vi "[ex ce] Handling Custom Data Types.vi"() -> ()   [LabVIEW 2021]
doc: "<B>Variable Manager example</B>\n\nThe VI demonstrates how to use user-defined data types with Variable Manager.\n\nThe VI generates a LabVIEW Waveform and saves it in a VarMan variable. The variable has a history attached, which saves every value written to the variable.\n\nThe example VI reads the variable to indicate current Waveform generated. Furthermore, it reads the variable history to indicate Waveforms generated recently.\n\n::: CalcExpress Toolkit :::\nCopyright (c) 2000-2026 Konstantin Shifershteyn. All rights reserved."
uses:
  <vilib>/measure/NI_MAPro.lvlib
panel:
  out "writerID":u32
  in  "tone phases":dbl[](array[numeric])=[137.63, 330.58, 66.37, 301.58] format="%.2p"
  in  "tone amplitudes":dbl[](array[numeric])=[2.0, 1.0, 1.0, 1.0] format="%.2p"
  in  "tone frequencies":dbl[](array[numeric])=[4.0, 2.0, 10.0, 8.0] format="%.2p"
  out "Timestamp":dbl format="%<%H:%M:%S%3u\n%x>T"
  in  "Hist Idx":i32(slide) caption="Historic point index" scale=0.0..99.0
  in  "Read History":bool
  out "Historic Graph":waveform(dbl)(graph)
  in  "stop":bool
  out "Waveform Graph":waveform(dbl)(graph)
  # "Review description for this VI and its Block Diagram for details"
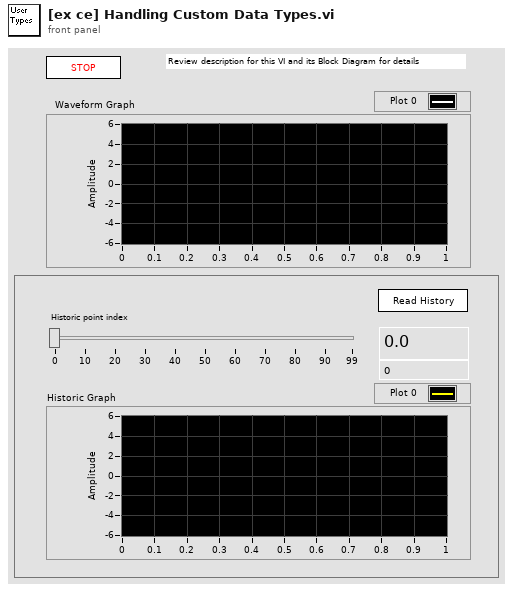
[diagram p1: front panel]
types:
  T1 = enum32{"nop", "create", "destroy", "reset", "get info", "config", "create_wrid"}
  T2 = typedef "VarMan Variable Context Handle.ctl" = i32
  T3 = enum8{"Enabled", "Disabled", "Disabled and Grayed Out"}
  T4 = typedef "VarMan Variable Data Statistics.ctl" = cluster{"writer ID":u32, "write MS":u32, "write TS":dbl, "write Cnt":u32}
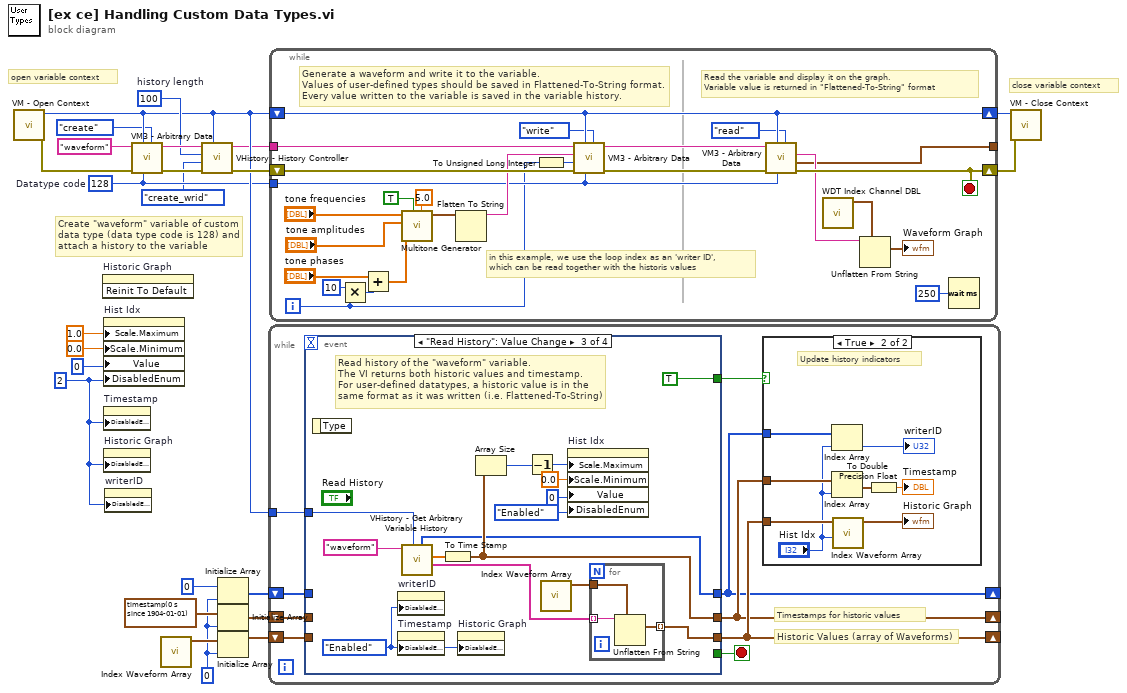
[diagram p0: block diagram]
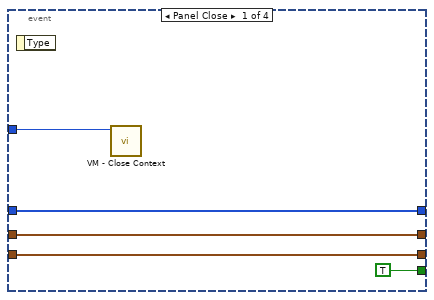
[diagram p3: hidden frame]
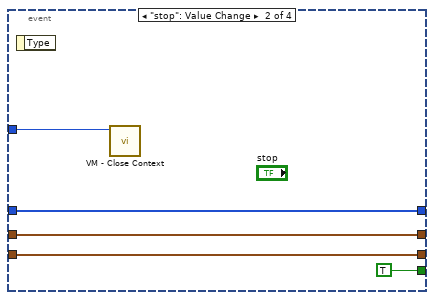
[diagram p4: hidden frame]
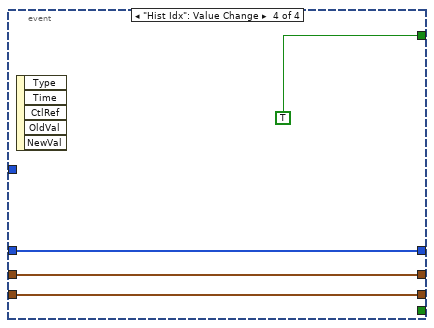
[diagram p5: hidden frame]
diagram:
  w4 = 0
  w19 = 100  # history length
  w1 = u8 2 ("Disabled")
  w14 = u32 128  # Datatype code
  # "close variable context"
  # "open variable context"
  # "Create \"waveform\" variable of custom\ndata type (data type code is 128) and\nattach a history to the variable"
  n1 = call "VM - Open Context.vi"() -> ("error out"=w23:errorcluster, "VC Handle out"=w16:T2)  [unwired: 9 in, 1 out]
  n2 = invoke on="Historic Graph" class="WFGraph (strict)" method="Reinit To Default"() -> ()  [unwired: 3 in, 3 out]
  n3 = property on="Hist Idx" class="Slide (strict)"("Scale.Maximum"=1.0 ("Scale.Range:Maximum"), "Scale.Minimum"=0.0 ("Scale.Range:Minimum"), "Value"=0 ("Slide"), "DisabledEnum"=w1) -> ()  [unwired: 2 in, 2 out]
  n4 = property on="Timestamp" class="DigNum (strict)"("DisabledEnum"=w1) -> ()  [unwired: 2 in, 2 out]
  n5 = property on="Historic Graph" class="WFGraph (strict)"("DisabledEnum"=w1) -> ()  [unwired: 2 in, 2 out]
  n6 = property on="writerID" class="DigNum (strict)"("DisabledEnum"=w1) -> ()  [unwired: 2 in, 2 out]
  n7 = call "VM3 - Arbitrary Data.vi"("cmd (read)"=enum16{"create", "destroy", "write", "read"}."create", "var type in"=w14, "VC Handle"=w16, "error in"=w23, "name_spec"="waveform" ("name")) -> ("error out"=w24:errorcluster, "dup name_spec"=w21:string)  [unwired: 2 in, 3 out]
  n8 = call-poly <vilib>:"Index Waveform Array.vi"() -> ("waveform"=w7:waveform(dbl))  [unwired: 10 in, 1 out]
  n9 = call "VHistory - History Controller.vi"("VC Handle"=w16, "error in"=w24, "cmd (nop:default)"=T1."create_wrid", "history length"=w19, "name_spec"=w21) -> ("error out"=w20:errorcluster, "dup name_spec"=w15:string)  [unwired: 3 in, 2 out]
  n10 = Initialize Array(u32 0, w4) -> (w3:u32[])
  n11 = Initialize Array(timestamp(0 s since 1904-01-01), w4) -> (w12:timestamp[])
  n12 = Initialize Array(w7, w4) -> (w13:waveform(dbl)[])
  n13 = while {
    tunnel: w16 -> [w33]
    shift-right: [w28] -> _
    shift-left: w13 -> [w32]
    shift-right: [w27] -> _
    shift-left: w12 -> [w31]
    shift-right: [w25] -> _
    shift-left: w3 -> [w26]
    stop <- w30 stop-if-true
    # "Timestamps for historic values"
    # "Historic Values (array of Waveforms)"
    n14 = event shown="[2] \"Read History\": Value Change" {
      selector: _ -> [_ _ _ _]
      dyn-events: _ -> [_ _ _ _]
      timeout: _ -> [_ _ _ _]
      tunnel: w33 -> [w44 w49 w66 _]
      tunnel: [w45 w50 w64 w73] -> w28
      tunnel: [w46 w51 w56 w72] -> w27
      tunnel: w32 -> [w45 w50 _ w73]
      tunnel: w31 -> [w46 w51 _ w72]
      tunnel: [TRUE TRUE _ _] -> w30
      tunnel: [_ _ TRUE TRUE] -> w29
      tunnel: [w42 w47 w53 w70] -> w25
      tunnel: w26 -> [w42 w47 _ w70]
      event Panel Close {
        n15 = event-data() -> ()  [unwired: 1 in, 1 out]
        n16 = call "VM - Close Context.vi"("VC Handle"=w44) -> ()  [unwired: 9 in, 2 out]
      }
      event "stop": Value Change {
        n17 = event-data() -> ()  [unwired: 1 in, 1 out]
        n18 = call "VM - Close Context.vi"("VC Handle"=w49) -> ()  [unwired: 9 in, 2 out]
      }
      event "Read History": Value Change {
        w52 = T3."Enabled" ("Disabled")
        # "Read history of the \"waveform\" variable.\nThe VI returns both historic values and timestamp.\nFor user-defined datatypes, a historic value is in the\nsame format as it was written (i.e. Flattened-To-String)"
        n19 = event-data() -> ()  [unwired: 1 in, 1 out]
        n20 = property on="writerID" class="DigNum (strict)"("DisabledEnum"=w52) -> ()  [unwired: 2 in, 2 out]
        n21 = property on="Timestamp" class="DigNum (strict)"("DisabledEnum"=w52) -> ()  [unwired: 2 in, 2 out]
        n22 = call "VHistory - Get Arbitrary Variable History.vi"("VC Handle"=w66, "name_spec"="waveform" ("name")) -> ("history"=w65:string[], "time stamps"=w63:dbl[], "writer IDs"=w53:u32[])  [unwired: 5 in, 2 out]
        n23 = To Time Stamp(1:w63) -> (0:w56:timestamp[])
        n24 = property on="Historic Graph" class="WFGraph (strict)"("DisabledEnum"=w52) -> ()  [unwired: 2 in, 2 out]
        n25 = Array Size(array=w56) -> (size(s)=w62:i32)
        n26 = Decrement(x=w62) -> (x-1=w58:i32)
        n27 = call-poly <vilib>:"Index Waveform Array.vi"() -> ("waveform"=w54:waveform(dbl))  [unwired: 10 in, 1 out]
        n28 = property on="Hist Idx" class="Slide (strict)"("Scale.Maximum"=w58, "Scale.Minimum"=0.0 ("Scale.Range:Minimum"), "Value"=0 ("Slide"), "DisabledEnum"=T3."Enabled" ("Disabled")) -> ()  [unwired: 2 in, 2 out]
        n29 = for {
          tunnel: w65 -> [w69] mode=indexing
          tunnel: w54 -> [w68]
          tunnel: [w67] -> w64 mode=indexing
          n30 = Unflatten From String(type=w68, binary string=w69) -> (value=w67:waveform(dbl))  [unwired: 3 in, 2 out]
        }
      }
      event "Hist Idx": Value Change {
        n31 = event-data() -> ()  [unwired: 1 in, 5 out]
      }
    }
    n32 = case shown="True" w29 {
      tunnel: w28 -> [_ w38]
      tunnel: w27 -> [_ w41]
      tunnel: w25 -> [_ w35]
      frame False {
      }
      frame True {
        # "Update history indicators"
        n33 = Index Array(array=w35, index="Hist Idx") -> (element=→"writerID":u32)
        n34 = Index Array(array=w41, index="Hist Idx") -> (element=w40:timestamp)
        n35 = call-poly <vilib>:"Index Waveform Array.vi"("index"="Hist Idx", "waveform array"=w38) -> ("waveform"=→"Historic Graph":waveform(dbl))  [unwired: 8 in, 1 out]
        n36 = To Double Precision Float(number=w40) -> (double precision float=→"Timestamp":dbl)
      }
    }
  }
  n37 = while {
    tunnel: w15 -> [w98]
    tunnel: w14 -> [w82]
    shift-right: [w85] -> w17
    shift-left: w20 -> [w97]
    shift-right: [w84] -> w18
    shift-left: w16 -> [w84]
    tunnel: [w76] -> _
    i -> [w75]
    stop <- w85 stop-if-true
    # "in this example, we use the loop index as an 'writer ID',\nwhich can be read together with the historis values"
    # "Read the variable and display it on the graph.\nVariable value is returned in \"Flattened-To-String\" format"
    # "Generate a waveform and write it to the variable.\nValues of user-defined types should be saved in Flattened-To-String format.\nEvery value written to the variable is saved in the variable history."
    n38 = Multiply(x=10, y=w75) -> (x*y=w89:i32)
    n39 = Add(x="tone phases", y=w89) -> (x+y=w91:dbl[])
    n40 = call <vilib>:"Multitone Generator.vi"("amplitude"=5.0, "reset signal"=TRUE, "tone phases"=w91, "tone amplitudes"="tone amplitudes", "tone frequencies"="tone frequencies") -> ("signal out"=w87:waveform(dbl))  [unwired: 3 in, 3 out]
    n41 = Flatten To String(anything=w87) -> (data string=w96:string)  [unwired: 3 in, 2 out]
    n42 = To Unsigned Long Integer(number=w75) -> (unsigned 32bit integer=w74:u32)
    n43 = call "VM3 - Arbitrary Data.vi"("cmd (read)"=enum16{"create", "destroy", "write", "read"}."write", "var type in"=w82, "VC Handle"=w84, "error in"=w97, "writer ID"=w74, "flattened value in"=w96, "name_spec"=w98) -> ("error out"=w86:errorcluster, "dup name_spec"=w83:string)  [unwired: 3 out]
    n44 = call "VM3 - Arbitrary Data.vi"("cmd (read)"=enum16{"create", "destroy", "write", "read"}."read", "var type in"=w82, "VC Handle"=w84, "error in"=w86, "name_spec"=w83) -> ("error out"=w85:errorcluster, "stats"=w76:T4, "flattened value out"=w81:string)  [unwired: 2 in, 2 out]
    n45 = call <vilib>:"WDT Index Channel DBL.vi"() -> ("waveform"=w80:waveform(dbl))  [unwired: 10 in, 1 out]
    n46 = Unflatten From String(type=w80, binary string=w81) -> (value=→"Waveform Graph":waveform(dbl))  [unwired: 3 in, 2 out]
    n47 = Wait (ms)(milliseconds to wait=u32 250) -> ()  [unwired: 1 out]
  }
  n48 = call "VM - Close Context.vi"("error in"=w17, "VC Handle"=w18) -> ()  [unwired: 8 in, 2 out]
